vi "test Verify Scripting Code.LUnit.approved.vi"   [LabVIEW 2020]
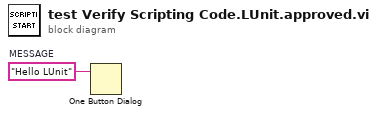
[diagram p0: block diagram]
diagram:
  w1 = "Hello LUnit"  # MESSAGE
  n1 = One Button Dialog(message=w1) -> ()  [unwired: 1 in, 1 out]
